vi "Read CTC100.vi"(8 "error in":errorcluster, 10 "Read channel":string, 11 "VISA resource name":refnum<visa-resource-name>) -> (0 "error out":errorcluster, 2 "Value out":dbl, 3 "VISA resource name out":refnum<visa-resource-name>)   [LabVIEW 2024]
uses:
  Simple VISA Reader/Simple VISA Reader Driver.lvclass
  GPIB/VISA  Send Receive.vi
panel:
  out "CTC channle name":string
  out "array":string[](array[string])
  in  "map":map{string, string}(c390)={"A"="In1", "B"="In2", "C"="In3", "D"="In4"}
  out "Outputs":string
  out "Output names":string
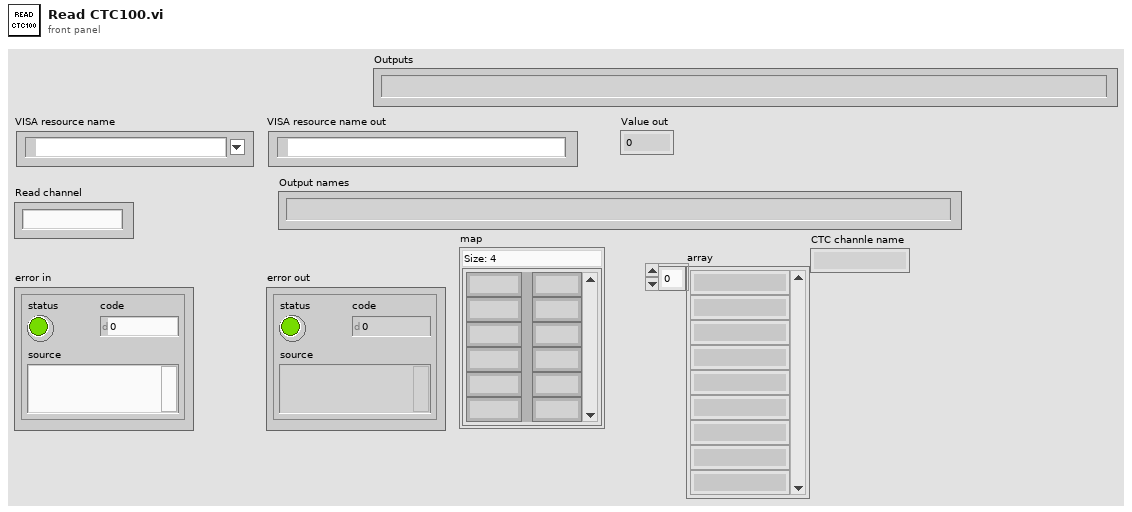
[diagram p1: front panel]
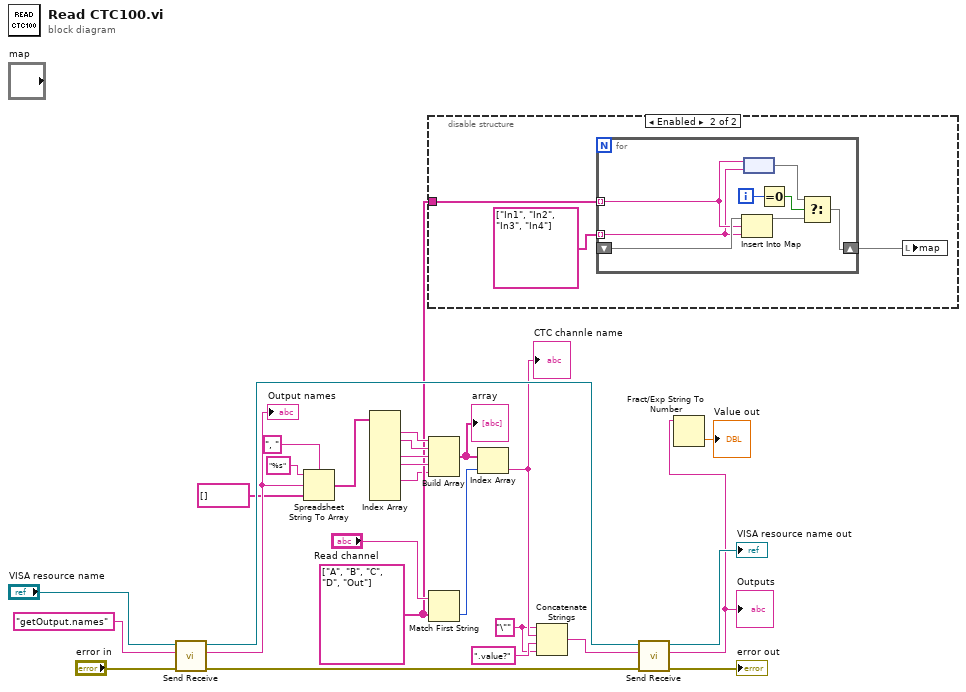
[diagram p0: block diagram]
diagram:
  w3 = "\""
  w10 = string[] ["A", "B", "C", "D", "Out"]
  n1 = call-poly "Send Receive.vi"("error in (no error)"="error in", "data string in"="getOutput.names", "VISA Resource Name"="VISA resource name") -> ("error out"=w21:errorcluster, "data string out"=w20:string, "VISA Resource Name Out"=w22:refnum<visa-resource-name>)  [unwired: 6 in]
  "Output names" <- w20
  n2 = Spreadsheet String To Array(delimiter (Tab)=", ", format string="%s", spreadsheet string=w20, array type (2D Dbl)=string[] []) -> (array=w15:string[])
  n3 = Index Array(array=w15) -> (element #1=w14:string, element #2=w13:string, element #4=w12:string, element #5=w11:string, element #7=w7:string)  [unwired: 9 in, 4 out]
  n4 = disable-structure shown="Enabled" {
    disable-tunnel: w10 -> [_ w28]
    frame Disabled {
    }
    frame Enabled {
      n5 = for {
        shift-right: [w33] -> w29
        shift-left: _ -> [w35]
        tunnel: w28 -> [w32] mode=indexing
        tunnel: string[] ["In1", "In2", "In3", "In4"] -> [w31] mode=indexing
        i -> [w38]
        n6 = Insert Into Map(map in=w35, key=w32, value=w31) -> (map out=w34:map{string, string})  [unwired: 2 out]
        n7 = node(w32, w31) -> (w36:map{string, string})
        n8 = Equal To 0?(x=w38) -> (x = 0?=w37:bool)
        n9 = Select(t=w36, s=w37, f=w34) -> (s? t:f=w33:map{string, string})
      }
      n10 = local write "map"(w29) -> ()
    }
  }
  n11 = Build Array(w14, w13, w12, w11, w7) -> (w8:string[])
  "array" <- w8
  n12 = Match First String(2:w10, 3:"Read channel") -> (0:w9:i32)  [unwired: 1 out]
  n13 = Index Array(array=w8, index=w9) -> (element=w5:string)
  "CTC channle name" <- w5
  n14 = Concatenate Strings(w3, w5, ".value?" ("data string in"), w3) -> (w6:string)
  n15 = call-poly "Send Receive.vi"("error in (no error)"=w21, "data string in"=w6, "VISA Resource Name"=w22) -> ("error out"=→"error out":errorcluster, "data string out"=w2:string, "VISA Resource Name Out"=→"VISA resource name out":refnum<visa-resource-name>)  [unwired: 6 in]
  "Outputs" <- w2
  n16 = Fract/Exp String To Number(string=w2) -> (number=→"Value out":dbl)  [unwired: 3 in, 1 out]
